vi "set Marker Type Map in Private Info.vi"(7 "All Off?":bool, 8 "error in (no error)":errorcluster, 9 "Marker Index":i32, 10 "Marker Mode":T1, 11 "FSV-40N in":refnum<class "FSV-40N.lvclass">) -> (0 "error out":errorcluster, 3 "FSV-40N out":refnum<class "FSV-40N.lvclass">)   [LabVIEW 2023, in "Spectrum Analyzer.lvlib" / "FSV-40N.lvclass"]
uses:
  FSV-40N.lvclass
  FSV-40N.lvclass/FSV-40N.ctl
  TYPE DEFINITION/TYPE Marker Control Mode.ctl
  Spectrum Analyzer.lvlib
  TYPE DEFINITION/TYPE Marker Type Map.ctl
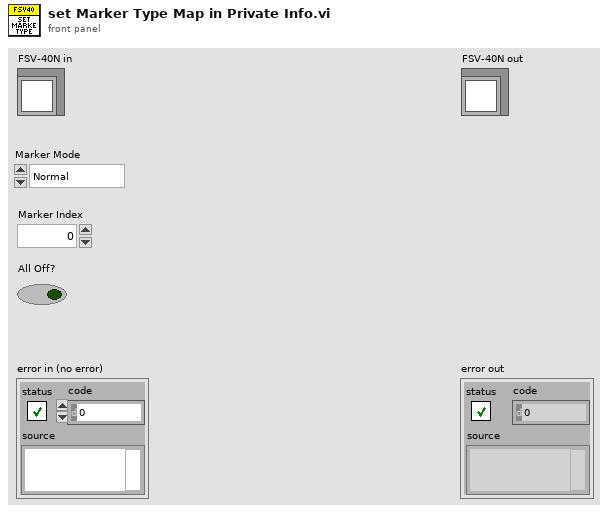
[diagram p1: front panel]
types:
  T1 = typedef "Spectrum Analyzer.lvlib/TYPE Marker Control Mode.ctl" = enum16{"Normal", "Delta", "Off"}
  T2 = typedef "Spectrum Analyzer.lvlib/TYPE Marker Type Map.ctl" = map{i32, T1}
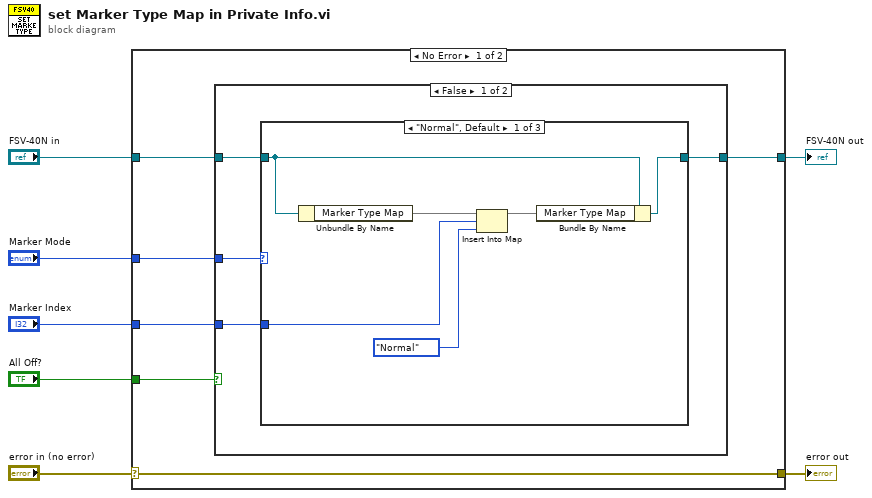
[diagram p0: block diagram]
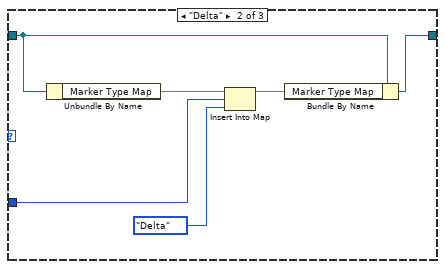
[diagram p2: hidden frame]
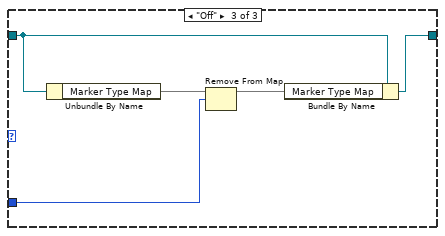
[diagram p3: hidden frame]
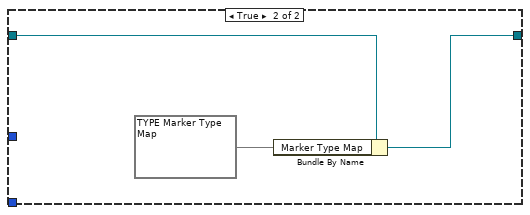
[diagram p4: hidden frame]
diagram:
  n1 = case shown="No Error" "error in (no error)" {
    selector: "error in (no error)" -> [w13 w39]
    tunnel: [w13 w39] -> w6
    tunnel: [w10 w38] -> w4
    tunnel: "FSV-40N in" -> [w11 w38]
    tunnel: "All Off?" -> [w12 _]
    tunnel: "Marker Mode" -> [w9 _]
    tunnel: "Marker Index" -> [w8 _]
    frame No Error {
      n2 = case shown="False" w12 {
        tunnel: w11 -> [w17 w37]
        tunnel: [w14 w35] -> w10
        tunnel: w9 -> [w16 _]
        tunnel: w8 -> [w15 _]
        frame False {
          n3 = case shown="\"Normal\", Default" w16 {
            tunnel: w17 -> [w20 w26 w34]
            tunnel: w15 -> [w22 w28 w31]
            tunnel: [w18 w24 w33] -> w14
            frame "Normal", Default {
              n4 = Unbundle By Name(w20) -> ("Marker Type Map"=w23:T2)
              n5 = Insert Into Map(map in=w23, key=w22, value=TYPE_Marker_Control_Mode."Normal") -> (map out=w19:T2)  [unwired: 2 out]
              n6 = Bundle By Name(cluster=w20, "Marker Type Map"=w19) -> (w18:refnum<class "FSV-40N.lvclass">)
            }
            frame "Delta" {
              n7 = Unbundle By Name(w26) -> ("Marker Type Map"=w29:T2)
              n8 = Insert Into Map(map in=w29, key=w28, value=TYPE_Marker_Control_Mode."Delta") -> (map out=w25:T2)  [unwired: 2 out]
              n9 = Bundle By Name(cluster=w26, "Marker Type Map"=w25) -> (w24:refnum<class "FSV-40N.lvclass">)
            }
            frame "Off" {
              n10 = Unbundle By Name(w34) -> ("Marker Type Map"=w32:T2)
              n11 = Remove From Map(10:w31, 11:w32) -> (3:w30:T2)  [unwired: 2 out]
              n12 = Bundle By Name(cluster=w34, "Marker Type Map"=w30) -> (w33:refnum<class "FSV-40N.lvclass">)
            }
          }
        }
        frame True {
          n13 = Bundle By Name(cluster=w37, "Marker Type Map"=T2 {}) -> (w35:refnum<class "FSV-40N.lvclass">)
        }
      }
    }
    frame Error {
    }
  }
  "error out" <- w6
  "FSV-40N out" <- w4
